vi "new_object.vi"() -> ()   [LabVIEW 2022 SP3]
uses:
  <vilib>/Utility/miscctls.llb/LVBoundsTypeDef.ctl
  <vilib>/Utility/miscctls.llb/LVPointTypeDef.ctl
panel:
  in  "style":u32
  out "object refnum":refnum<vi>
  out "error out":errorcluster
  in  "owner refnum":refnum<vi>
  in  "location":T1
  in  "error in (no error)":errorcluster
  in  "auto wire? (F)":bool
  in  "bounds":T2
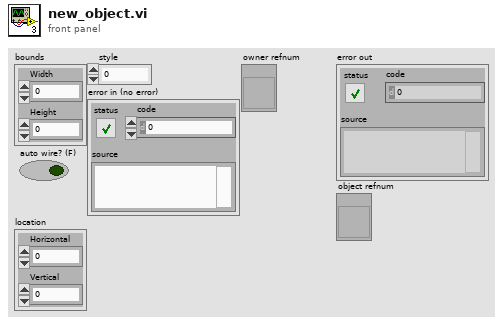
[diagram p1: front panel]
types:
  T1 = typedef "LVPointTypeDef.ctl" = cluster{"Horizontal":i16, "Vertical":i16}
  T2 = typedef "LVBoundsTypeDef.ctl" = cluster{"Width":u32, "Height":u32}
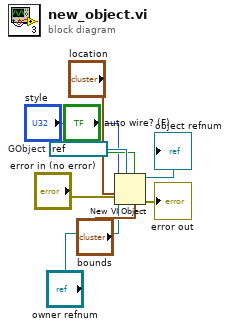
[diagram p0: block diagram]
diagram:
  w9 = refnum<vi> refnum  # GObject
  n1 = New VI Object(vi object class=w9, auto wire? (F)="auto wire? (F)", owner refnum="owner refnum", style="style", position/next to="location", 4:"bounds", 8:"error in (no error)") -> (object refnum=→"object refnum":refnum<vi>, 0:→"error out":errorcluster)  [unwired: 1 in]
